vi "process.vi"(8 "error in (no error)":errorcluster, 11 "Subscription in":refnum<class "_Subscription.lvclass">) -> ()   [LabVIEW 2013, in "MQTT Server.lvlib" / "_Subscription.lvclass"]
uses:
  _Subscription.lvclass
  <vilib>/LabVIEW Open Source Project/MQTT Control Packets/Control Packets/ControlPacket/QualityOfService -- enum.ctl
  _Subscription.lvclass/_Subscription.ctl
  TopicFilter/_TopicFilter.lvclass/_TopicFilter.ctl
  <vilib>/LabVIEW Open Source Project/MQTT Control Packets/Control Packets/Ack/Ack.lvclass
  <vilib>/LabVIEW Open Source Project/MQTT Control Packets/Control Packets/PUBLISH/PUBLISH.lvclass
  <vilib>/LabVIEW Open Source Project/MQTT Control Packets/Control Packets/ControlPacket/ControlPacket.lvclass/ControlPacket.ctl
  <vilib>/LabVIEW Open Source Project/MQTT Control Packets/Control Packets/ControlPacket/ControlPacket.lvclass
panel:
  out "QoS":T1
  out "Topic Filter":string
  out "Numeric":i32
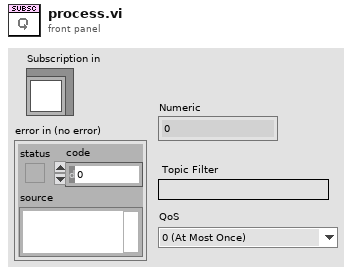
[diagram p1: front panel]
types:
  T1 = typedef "MQTT_Control_Packets.lvlib/ControlPacket.lvclass/QualityOfService -- enum.ctl" = enum16{"0 (At Most Once)", "1 (At Least Once)", "2 (Exactly Once)"}
  T2 = typedef "MQTT Server.lvlib/_Subscription.lvclass/Stored Packet -- cluster.ctl" = cluster{"Packet Identifier":u16, "ControlPacket":refnum<class "ControlPacket.lvclass">, "last attempt":timestamp}
  T3 = typedef "MQTT_Control_Packets.lvlib/ControlPacket.lvclass/Control Packet Type -- enum.ctl" = enum16{"Reserved", "CONNECT", "CONNACK", "PUBLISH", "PUBACK", "PUBREC", "PUBREL", "PUBCOMP", "SUBSCRIBE", "SUBACK", "UNSUBSCRIBE", "UNSUBACK", "PINGREQ", "PINGRESP", "DISCONNECT", "AUTH"}
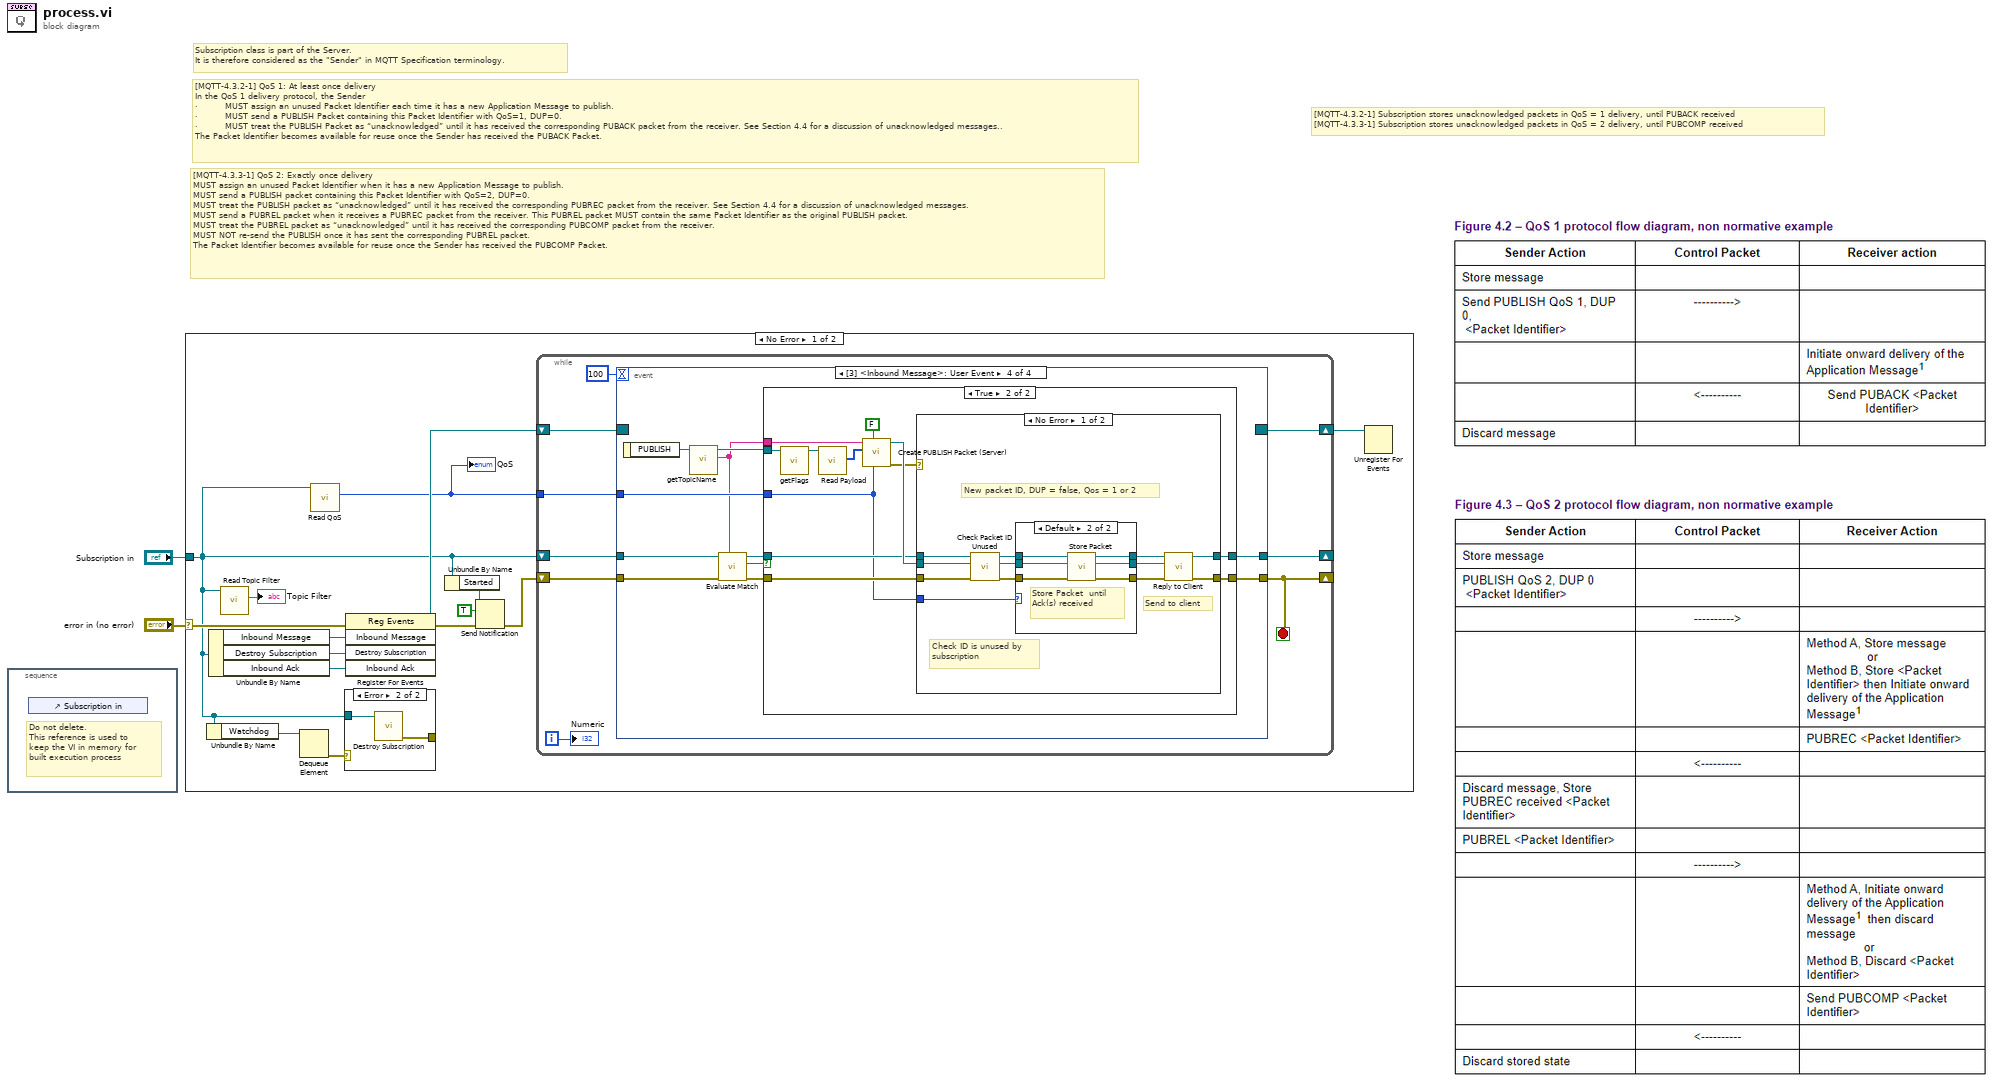
[diagram p0: block diagram]
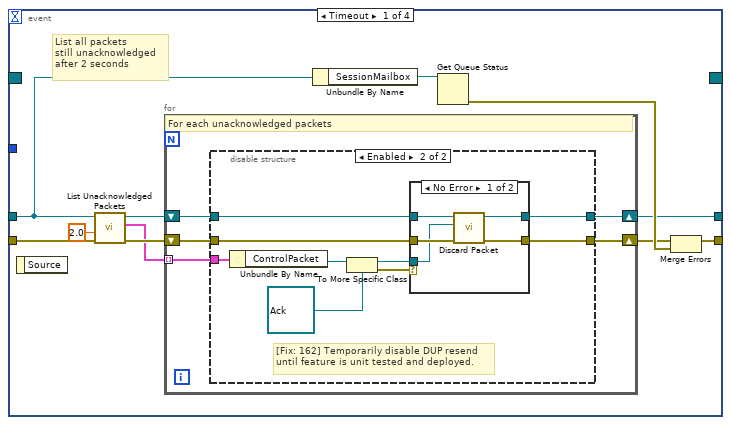
[diagram p3: hidden frame]
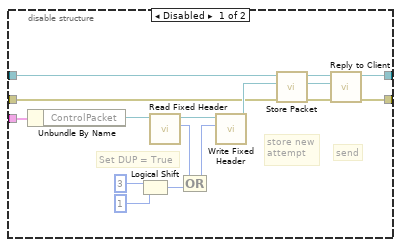
[diagram p4: hidden frame]
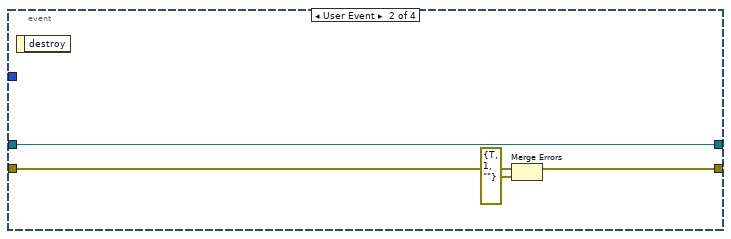
[diagram p6: hidden frame]
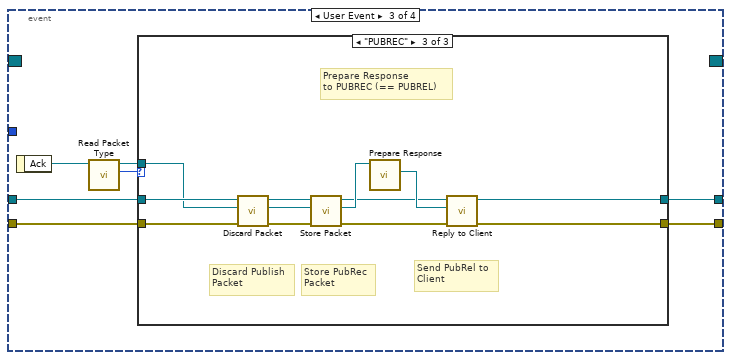
[diagram p7: hidden frame]
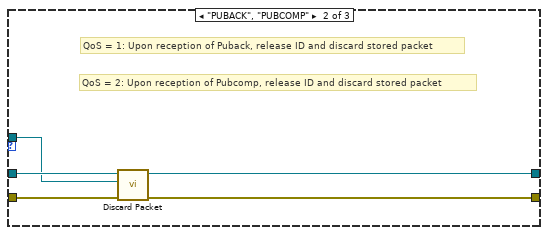
[diagram p9: hidden frame]
diagram:
  # "[MQTT-4.3.2-1] Subscription stores unacknowledged packets in QoS = 1 delivery, until PUBACK received\n[MQTT-4.3.3-1] Subscription stores unacknowledged packets in QoS = 2 delivery, until PUBCOMP received"
  # "[MQTT-4.3.3-1] QoS 2: Exactly once delivery\nMUST assign an unused Packet Identifier when it has a new Application Message to publish.\nMUST send a PUBLISH packet containing this Packet Identifier with QoS=2, DUP=0.\nMUST treat the PUBLISH packet as “unacknowledged” until it has received the corresponding PUBREC packet from the receiver. See Section 4.4 for a discussion of unacknowledged messages.\nMUST send a PUBREL packet when it receives a PUBREC packet from the receiver. This PUBREL packet MUST contain the same Packet Identifier as the original PUBLISH packet.\nMUST treat the PUBREL packet as “unacknowledged” until it has received the corresponding PUBCOMP packet from the receiver.\nMUST NOT re-send the PUBLISH once it has sent the corresponding PUBREL packet.\nThe Packet Identifier becomes available for reuse once the Sender has received the PUBCOMP Packet."
  # "[MQTT-4.3.2-1] QoS 1: At least once delivery\nIn the QoS 1 delivery protocol, the Sender\n·         MUST assign an unused Packet Identifier each time it has a new Application Message to publish.\n·         MUST send a PUBLISH Packet containing this Packet Identifier with QoS=1, DUP=0.\n·         MUST treat the PUBLISH Packet as “unacknowledged” until it has received the corresponding PUBACK packet from the receiver. See Section 4.4 for a discussion of unacknowledged messages..\nThe Packet Identifier becomes available for reuse once the Sender has received the PUBACK Packet."
  # "Subscription class is part of the Server.\nIt is therefore considered as the \"Sender\" in MQTT Specification terminology."
  n1 = stacked-sequence {
    frame #0 {
      # "Do not delete.\nThis reference is used to keep the VI in memory for built execution process"
      n2 = control-ref of="Subscription in"() -> ()  [unwired: 1 out]
    }
  }
  n3 = case shown="No Error" "error in (no error)" {
    selector: "error in (no error)" -> [w15 _]
    tunnel: "Subscription in" -> [w4 _]
    frame No Error {
      n4 = Unbundle By Name(w4) -> ("Watchdog"=w10:refnum<queue>)
      n5 = Unbundle By Name(w4) -> ("Inbound Message"=w8:refnum<user-event>, "Destroy Subscription"=w7:refnum<user-event>, "Inbound Ack"=w5:refnum<user-event>)
      n6 = call "Read Topic Filter.vi"("Subscription in"=w4) -> ("Topic Filter"=→"Topic Filter":string)  [unwired: 7 in, 3 out]
      n7 = Dequeue Element(queue=w10) -> (error out=w9:errorcluster)  [unwired: 2 in, 3 out]
      n8 = call "Read QoS.vi"("Subscription in"=w4) -> ("QoS"=w3:T1)  [unwired: 8 in, 2 out]
      "QoS" <- w3
      n9 = case shown="Error" w9 {
        tunnel: w4 -> [_ w19]
        tunnel: [_ w18] -> _
        frame No Error {
        }
        frame Error {
          n10 = call "Destroy Subscription.vi"("Subscription in"=w19) -> ("error out"=w18:errorcluster)  [unwired: 9 in, 1 out]
        }
      }
      n11 = register-events(error in=w15, w8, w7, w5) -> (reference out=w13:refnum<event-registration>, error out=w14:errorcluster)  [unwired: 1 in]
      n12 = Unbundle By Name(w4) -> ("Started"=w6:refnum<notifier>)
      n13 = Send Notification(notification=TRUE, notifier=w6, error in (no error)=w14) -> (error out=w16:errorcluster)  [unwired: 1 out]
      n14 = while {
        shift-right: [w24] -> _
        shift-left: w16 -> [w20]
        shift-right: [w26] -> w12
        shift-left: w13 -> [w27]
        shift-right: [w22] -> _
        shift-left: w4 -> [w25]
        tunnel: w3 -> [w21]
        i -> [w23]
        stop <- w24 stop-if-true
        n15 = event shown="[3] <Inbound Message>: User Event" {
          selector: w27 -> [_ _ _ _]
          dyn-events: [_ _ _ _] -> w26
          timeout: 100 -> [_ _ _ _]
          tunnel: w25 -> [w36 w79 w85 w110]
          tunnel: [w37 w80 w81 w117] -> w24
          tunnel: [w32 w79 w82 w112] -> w22
          tunnel: w21 -> [_ _ _ w108]
          tunnel: w20 -> [w35 w77 w84 w109]
          event Timeout {
            # "List all packets\nstill unacknowledged\nafter 2 seconds"
            n16 = event-data() -> ()  [unwired: 1 in, 1 out]
            n17 = call "List Unacknowledged Packets.vi"("error in (no error)"=w35, "filter (0s: list all)"=2.0, "Subscription in"=w36) -> ("error out"=w31:errorcluster, "Unacknowledged"=w29:T2[], "Subscription out"=w33:refnum<class "_Subscription.lvclass">)  [unwired: 6 in]
            n18 = for {
              shift-right: [w43] -> w32
              shift-left: w33 -> [w41]
              shift-right: [w42] -> w30
              shift-left: w31 -> [w40]
              tunnel: w29 -> [w44] mode=indexing
              # "For each unacknowledged packets"
              n19 = disable-structure shown="Enabled" {
                disable-tunnel: w44 -> [w60 w69]
                disable-tunnel: [w52 w67] -> w43
                disable-tunnel: [w51 w66] -> w42
                disable-tunnel: w41 -> [w50 w68]
                disable-tunnel: w40 -> [w46 w65]
                frame Disabled {
                  # "send"
                  # "store new\nattempt"
                  # "Set DUP = True"
                  n20 = Unbundle By Name(w60) -> ("ControlPacket"=w55:refnum<class "ControlPacket.lvclass">)
                  n21 = Logical Shift(y=i16 3, x=u8 1) -> (x << y=w56:u8)
                  n22 = call <vilib>:"Read Fixed Header.vi"("ControlPacket in"=w55) -> ("Fixed Header"=w54:u8, "ControlPacket out"=w59:refnum<class "ControlPacket.lvclass">)  [unwired: 9 in]
                  n23 = Compound Arithmetic op=OR(w54, w56) -> (w53:u8)
                  n24 = call <vilib>:"Write Fixed Header.vi"("Fixed Header"=w53, "ControlPacket in"=w59) -> ("ControlPacket out"=w48:refnum<class "ControlPacket.lvclass">)  [unwired: 9 in]
                  n25 = call "Store Packet.vi"("error in (no error)"=w46, "ControlPacket"=w48, "Subscription in"=w50) -> ("error out"=w45:errorcluster, "ControlPacket dup"=w47:refnum<class "ControlPacket.lvclass">, "Subscription out"=w49:refnum<class "_Subscription.lvclass">)  [unwired: 6 in]
                  n26 = call "Reply to Client.vi"("error in (no error)"=w45, "ControlPacket"=w47, "Subscription in"=w49) -> ("error out"=w51:errorcluster, "Subscription out"=w52:refnum<class "_Subscription.lvclass">)  [unwired: 7 in]
                }
                frame Enabled {
                  # "[Fix: 162] Temporarily disable DUP resend\nuntil feature is unit tested and deployed."
                  n27 = Unbundle By Name(w69) -> ("ControlPacket"=w64:refnum<class "ControlPacket.lvclass">)
                  n28 = To More Specific Class(target class=refnum<class "Ack.lvclass"> refnum ("Ack"), reference=w64) -> (specific class reference=w61:refnum<class "Ack.lvclass">, error out=w62:errorcluster)  [unwired: 1 in]
                  n29 = case shown="No Error" w62 {
                    tunnel: w68 -> [w74 w76]
                    tunnel: [w73 w76] -> w67
                    tunnel: [w72 w75] -> w66
                    tunnel: w65 -> [w71 w75]
                    tunnel: w61 -> [w70 _]
                    frame No Error {
                      n30 = call "Discard Packet.vi"("error in (no error)"=w71, "Ack"=w70, "Subscription in"=w74) -> ("error out"=w72:errorcluster, "Subscription out"=w73:refnum<class "_Subscription.lvclass">)  [unwired: 5 in, 2 out]
                    }
                    frame Error {
                    }
                  }
                }
              }
            }
            n31 = Unbundle By Name(w36) -> ("SessionMailbox"=w39:refnum<queue>)
            n32 = Get Queue Status(queue=w39) -> (error out=w38:errorcluster)  [unwired: 2 in, 7 out]
            n33 = Merge Errors(w30, w38) -> (w37:errorcluster)
          }
          event User Event {
            n34 = event-data() -> ()  [unwired: 1 in, 1 out]
            n35 = Merge Errors(w77, errorcluster {"status"=TRUE, "code"=1, "source"=""} ("error in")) -> (w80:errorcluster)
          }
          event User Event {
            n36 = event-data() -> ("Ack"=w87:refnum<class "Ack.lvclass">)  [unwired: 1 in]
            n37 = call <vilib>:"Read Packet Type.vi"("ControlPacket in"=w87) -> ("Control Packet Type"=w86:T3, "ControlPacket out"=w83:refnum<class "Ack.lvclass">)  [unwired: 9 in]
            n38 = case shown="\"PUBREC\"" w86 {
              tunnel: w85 -> [w89 w94 w106]
              tunnel: w84 -> [w88 w92 w104]
              tunnel: w83 -> [_ w93 w105]
              tunnel: [w89 w91 w97] -> w82
              tunnel: [w88 w90 w95] -> w81
              frame Default {
                # "Already discarded packets.\nDuplicates ==> ignore"
              }
              frame "PUBACK", "PUBCOMP" {
                # "QoS = 2: Upon reception of Pubcomp, release ID and discard stored packet"
                # "QoS = 1: Upon reception of Puback, release ID and discard stored packet"
                n39 = call "Discard Packet.vi"("error in (no error)"=w92, "Ack"=w93, "Subscription in"=w94) -> ("error out"=w90:errorcluster, "Subscription out"=w91:refnum<class "_Subscription.lvclass">)  [unwired: 5 in, 2 out]
              }
              frame "PUBREC" {
                # "Prepare Response\nto PUBREC (== PUBREL)"
                # "Send PubRel to\nClient"
                # "Store PubRec\nPacket"
                # "Discard Publish\nPacket"
                n40 = call "Discard Packet.vi"("error in (no error)"=w104, "Ack"=w105, "Subscription in"=w106) -> ("error out"=w101:errorcluster, "Ack dup"=w102:refnum<class "Ack.lvclass">, "Subscription out"=w103:refnum<class "_Subscription.lvclass">)  [unwired: 5 in, 1 out]
                n41 = call "Store Packet.vi"("error in (no error)"=w101, "ControlPacket"=w102, "Subscription in"=w103) -> ("error out"=w96:errorcluster, "ControlPacket dup"=w100:refnum<class "Ack.lvclass">, "Subscription out"=w98:refnum<class "_Subscription.lvclass">)  [unwired: 6 in]
                n42 = call-dynamic "Prepare Response.vi"("ControlPacket in"=w100) -> ("ControlPacket response"=w99:refnum<class "ControlPacket.lvclass">)  [unwired: 7 in, 3 out]
                n43 = call "Reply to Client.vi"("error in (no error)"=w96, "ControlPacket"=w99, "Subscription in"=w98) -> ("error out"=w95:errorcluster, "Subscription out"=w97:refnum<class "_Subscription.lvclass">)  [unwired: 7 in]
              }
            }
          }
          event User Event {
            n44 = event-data() -> ("PUBLISH"=w111:refnum<class "PUBLISH.lvclass">)  [unwired: 1 in]
            n45 = call <vilib>:"getTopicName.vi"("PUBLISH in"=w111) -> ("Topic"=w107:string, "PUBLISH out"=w116:refnum<class "PUBLISH.lvclass">)  [unwired: 8 in, 1 out]
            n46 = call "Evaluate Match.vi"("Topic"=w107, "error in (no error)"=w109, "Subscription in"=w110) -> ("error out"=w113:errorcluster, "Matched"=w115:bool, "Subscription out"=w114:refnum<class "_Subscription.lvclass">)  [unwired: 5 in, 1 out]
            n47 = case shown="True" w115 {
              tunnel: [w119 w131] -> w117
              tunnel: w113 -> [w119 w126]
              tunnel: w114 -> [w118 w124]
              tunnel: w116 -> [_ w123]
              tunnel: [w118 w130] -> w112
              tunnel: w107 -> [_ w129]
              tunnel: w108 -> [_ w121]
              frame False {
                # "Not a match for subscription"
              }
              frame True {
                n48 = call-dynamic "getFlags.vi"("PUBLISH in"=w123) -> ("PUBLISH out"=w122:refnum<class "PUBLISH.lvclass">)  [unwired: 7 in, 3 out]
                n49 = call <vilib>:"Read Payload.vi"("ControlPacket in"=w122) -> ("Payload"=w127:u8[])  [unwired: 9 in, 1 out]
                n50 = call <vilib>:"Create PUBLISH Packet (Server).vi"("QoS"=w121, "DUP (Re-delivery attempt)"=FALSE, "Payload"=w127, "Topic Name"=w129) -> ("error out"=w120:errorcluster, "PUBLISH"=w125:refnum<class "PUBLISH.lvclass">)  [unwired: 4 in, 2 out]
                n51 = case shown="No Error" w120 {
                  tunnel: [w143 w153] -> w131
                  tunnel: [w142 w154] -> w130
                  tunnel: w126 -> [w138 w153]
                  tunnel: w125 -> [w136 _]
                  tunnel: w124 -> [w134 w154]
                  tunnel: w121 -> [w132 _]
                  frame No Error {
                    # "New packet ID, DUP = false, Qos = 1 or 2"
                    # "Send to client"
                    # "Check ID is unused by\nsubscription"
                    n52 = call "Check Packet ID Unused.vi"("error in (no error)"=w138, "PUBLISH"=w136, "Subscription in"=w134) -> ("error out"=w137:errorcluster, "PUBLISH out"=w135:refnum<class "PUBLISH.lvclass">, "Subscription out"=w133:refnum<class "_Subscription.lvclass">)  [unwired: 6 in]
                    n53 = case shown="Default" w132 {
                      tunnel: w133 -> [w146 w152]
                      tunnel: [w146 w151] -> w141
                      tunnel: [w145 w148] -> w140
                      tunnel: w137 -> [w145 w149]
                      tunnel: w135 -> [w144 w150]
                      tunnel: [w144 w147] -> w139
                      frame "0 (At Most Once)" {
                      }
                      frame Default {
                        # "Store Packet  until Ack(s) received"
                        n54 = call "Store Packet.vi"("error in (no error)"=w149, "ControlPacket"=w150, "Subscription in"=w152) -> ("error out"=w148:errorcluster, "ControlPacket dup"=w147:refnum<class "PUBLISH.lvclass">, "Subscription out"=w151:refnum<class "_Subscription.lvclass">)  [unwired: 6 in]
                      }
                    }
                    n55 = call "Reply to Client.vi"("error in (no error)"=w140, "ControlPacket"=w139, "Subscription in"=w141) -> ("error out"=w143:errorcluster, "Subscription out"=w142:refnum<class "_Subscription.lvclass">)  [unwired: 7 in]
                  }
                  frame Error {
                    # "Invalidly built packet"
                  }
                }
              }
            }
          }
        }
        "Numeric" <- w23
      }
      n56 = Unregister For Events(event registration refnum=w12) -> ()  [unwired: 1 in, 1 out]
    }
    frame Error {
    }
  }
